vi "Load SA Range Setting.vi"(8 "error in (no error)":errorcluster caption="에러 입력(에러 없음)", 10 "SA Range Param":T1, 11 "Instrument Manager 입력":refnum<class "Instrument Manager.lvclass">) -> (0 "error out":errorcluster caption="에러 출력", 3 "Instrument Manager 출력":refnum<class "Instrument Manager.lvclass">)   [LabVIEW 2023, in "Instrument Manager.lvclass"]
uses:
  Instrument Manager.lvclass
  Instrument Manager.lvclass/Instrument Manager.ctl
  Module/Spectrum Analyzer/TYPE DEFINITION/TYPE Display Trace Mode Select.ctl
  Module/Spectrum Analyzer/Spectrum Analyzer.lvlib
  f5ec1ae0-98d7-4c12-bcf4-21a1374e48ca.vi
  Module/Spectrum Analyzer/TYPE DEFINITION/TYPE Detect Mode Select.ctl
  Type Definition/SA Range Param.ctl
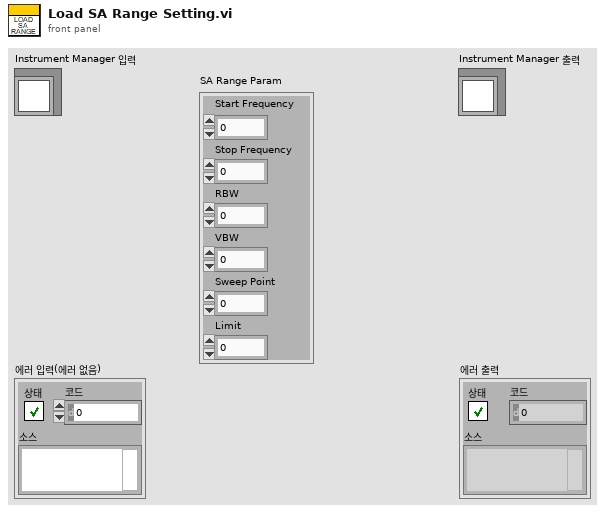
[diagram p1: front panel]
types:
  T1 = typedef "SA Range Param.ctl" = cluster{"Start Frequency":dbl, "Stop Frequency":dbl, "RBW":dbl, "VBW":dbl, "Sweep Point":u32, "Limit":dbl}
  T2 = typedef "Spectrum Analyzer.lvlib/TYPE Display Trace Mode Select.ctl" = enum16{"Clear Write", "Max Hold", "Min Hold", "Average", "View"}
  T3 = typedef "Spectrum Analyzer.lvlib/TYPE Detect Mode Select.ctl" = enum16{"Det Auto (Normal)", "Auto Peak", "Positive Peak", "Negative Peak", "Sample", "RMS", "Average", "Quasipeak", "CISPR Average", "RMS Average"}
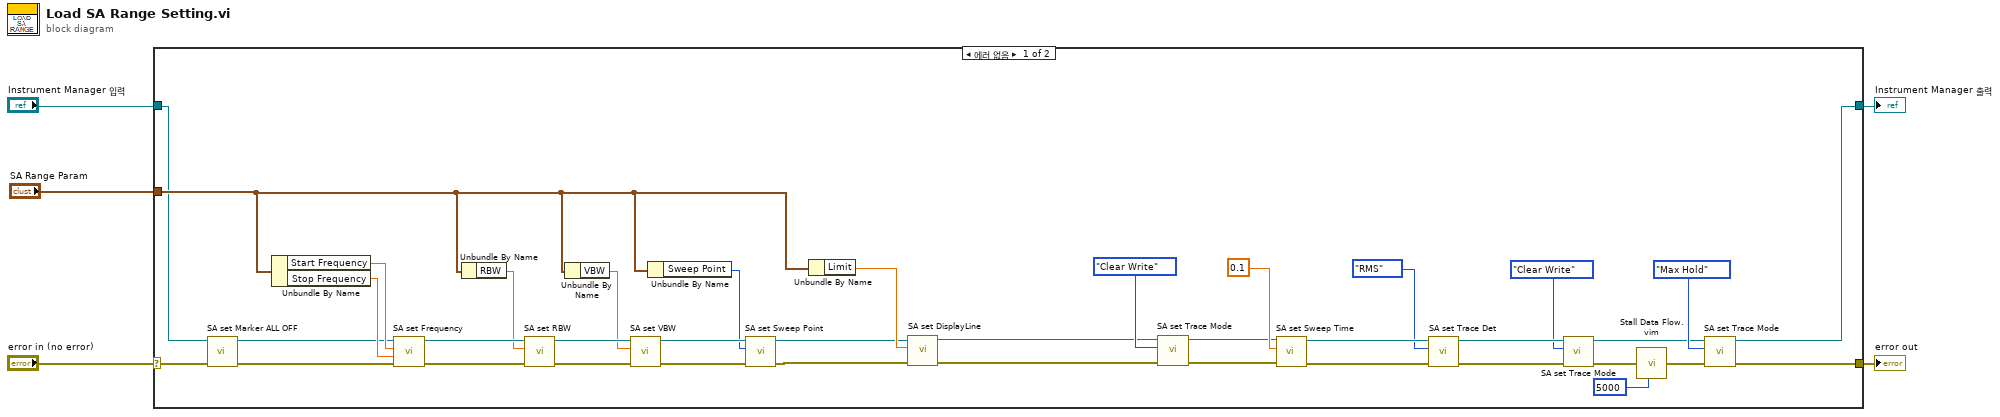
[diagram p0: block diagram]
diagram:
  n1 = case shown="에러 없음" "error in (no error)" {
    selector: "error in (no error)" -> [w9 w45]
    tunnel: [w37 w45] -> w4
    tunnel: [w36 w44] -> w2
    tunnel: "Instrument Manager 입력" -> [w7 w44]
    tunnel: "SA Range Param" -> [w15 _]
    frame No Error {
      n2 = call "SA set Marker ALL OFF.vi"("error in (no error)"=w9, "Instrument Manager 입력"=w7) -> ("error out"=w8:errorcluster, "Instrument Manager 출력"=w6:refnum<class "Instrument Manager.lvclass">)  [unwired: 8 in]
      n3 = Unbundle By Name(w15) -> ("Start Frequency"=w34:dbl, "Stop Frequency"=w35:dbl)
      n4 = call "SA set Frequency.vi"("error in (no error)"=w8, "Stop"=w35, "Start"=w34, "Instrument Manager 입력"=w6) -> ("error out"=w43:errorcluster, "Instrument Manager 출력"=w40:refnum<class "Instrument Manager.lvclass">)  [unwired: 6 in]
      n5 = Unbundle By Name(w15) -> ("RBW"=w33:dbl)
      n6 = call "SA set RBW.vi"("error in (no error)"=w43, "BW Value (Hz)"=w33, "Instrument Manager 입력"=w40) -> ("error out"=w42:errorcluster, "Instrument Manager 출력"=w39:refnum<class "Instrument Manager.lvclass">)  [unwired: 7 in]
      n7 = Unbundle By Name(w15) -> ("VBW"=w32:dbl)
      n8 = call "SA set VBW.vi"("error in (no error)"=w42, "BW Value (Hz)"=w32, "Instrument Manager 입력"=w39) -> ("error out"=w41:errorcluster, "Instrument Manager 출력"=w38:refnum<class "Instrument Manager.lvclass">)  [unwired: 7 in]
      n9 = Unbundle By Name(w15) -> ("Sweep Point"=w31:u32)
      n10 = call "SA set Sweep Point.vi"("error in (no error)"=w41, "Sweep Point"=w31, "Instrument Manager 입력"=w38) -> ("error out"=w13:errorcluster, "Instrument Manager 출력"=w11:refnum<class "Instrument Manager.lvclass">)  [unwired: 7 in]
      n11 = Unbundle By Name(w15) -> ("Limit"=w14:dbl)
      n12 = call "SA set DisplayLine.vi"("error in (no error)"=w13, "Amplitude"=w14, "Instrument Manager 입력"=w11) -> ("error out"=w12:errorcluster, "Instrument Manager 출력"=w10:refnum<class "Instrument Manager.lvclass">)  [unwired: 7 in]
      n13 = call "SA set Trace Mode.vi"("error in (no error)"=w12, "Trace Mode"=TYPE_Display_Trace_Mode_Select."Clear Write", "Instrument Manager 입력"=w10) -> ("error out"=w17:errorcluster, "Instrument Manager 출력"=w18:refnum<class "Instrument Manager.lvclass">)  [unwired: 7 in]
      n14 = call "SA set Sweep Time.vi"("error in (no error)"=w17, "Sweep Time(sec)"=0.1, "Instrument Manager 입력"=w18) -> ("error out"=w29:errorcluster, "Instrument Manager 출력"=w26:refnum<class "Instrument Manager.lvclass">)  [unwired: 7 in]
      n15 = call "SA set Trace Det.vi"("error in (no error)"=w29, "Detector Type"=TYPE_Detect_Mode_Select."RMS", "Instrument Manager 입력"=w26) -> ("error out"=w28:errorcluster, "Instrument Manager 출력"=w27:refnum<class "Instrument Manager.lvclass">)  [unwired: 7 in]
      n16 = call "SA set Trace Mode.vi"("error in (no error)"=w28, "Trace Mode"=TYPE_Display_Trace_Mode_Select."Clear Write", "Instrument Manager 입력"=w27) -> ("error out"=w21:errorcluster, "Instrument Manager 출력"=w22:refnum<class "Instrument Manager.lvclass">)  [unwired: 7 in]
      n17 = call "Stall Data Flow.vim"("value in"=w21, "milliseconds to wait"=u32 5000) -> ("value out"=w20:errorcluster)  [unwired: 1 out]
      n18 = call "SA set Trace Mode.vi"("error in (no error)"=w20, "Trace Mode"=TYPE_Display_Trace_Mode_Select."Max Hold", "Instrument Manager 입력"=w22) -> ("error out"=w37:errorcluster, "Instrument Manager 출력"=w36:refnum<class "Instrument Manager.lvclass">)  [unwired: 7 in]
    }
    frame Error {
    }
  }
  "error out" <- w4
  "Instrument Manager 출력" <- w2
